vi "Register.vi"(4 "line limit":i32, 6 "log limit":i32, 8 "error in (no error)":errorcluster, 9 "auto-scroll":bool, 10 "ctl ref":refnum<vi>, 11 "handler name":string) -> (0 "error out":errorcluster)   [LabVIEW 2018, in "GLog.lvlib" / "UI Updater.lvlib"]
uses:
  UI Updater.lvlib
  UI Updater.vi
  UI Updater Global.vi
panel:
  # "Connector Pane"
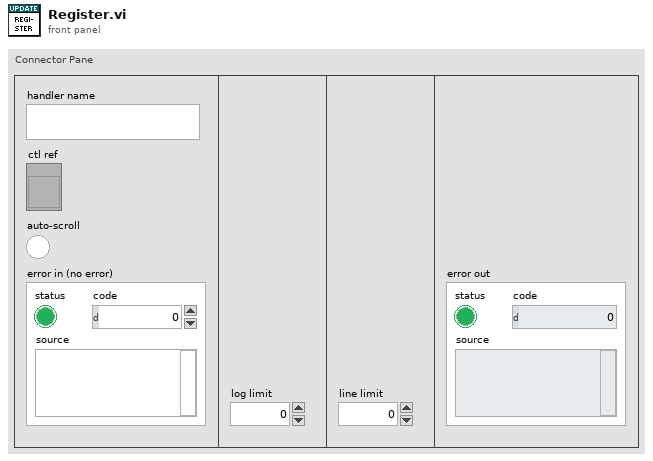
[diagram p1: front panel]
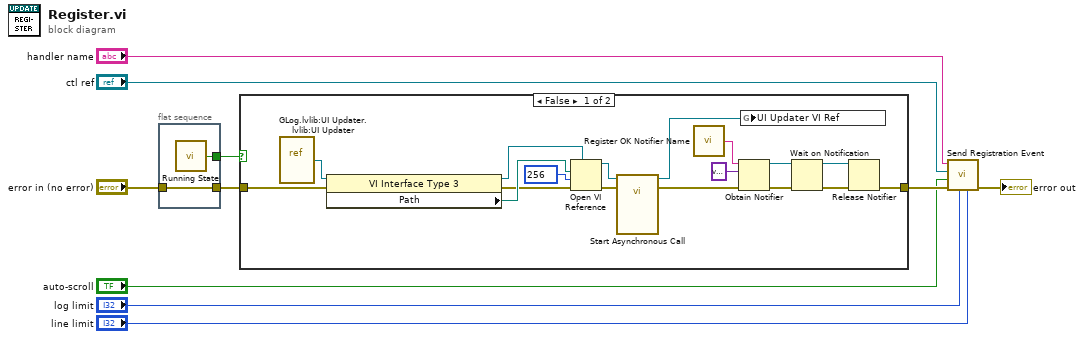
[diagram p0: block diagram]
diagram:
  n1 = flat-sequence {
    tunnel: [w12] -> w10
    tunnel: [w11] -> w2
    tunnel: "error in (no error)" -> [w11]
    frame #0 {
      n2 = call "Running State.vi"() -> ("Running?"=w12:bool)  [unwired: 1 in]
    }
  }
  n3 = case shown="False" w10 {
    tunnel: [w15 w30] -> w9
    tunnel: w2 -> [w22 w30]
    frame False {
      n4 = vi-ref "GLog.lvlib:UI Updater.lvlib:UI Updater.vi"() -> (w27:refnum<vi>)
      n5 = property class="VI Interface Type 3"(reference=w27, error in=w22) -> (reference out=w26:refnum<vi>, error out=w23:errorcluster, "Path"=w28:path)
      n6 = Open VI Reference(type specifier VI Refnum (for type only)=w26, vi path=w28, options=256, error in (no error)=w23) -> (vi reference=w29:refnum<vi>, error out=w24:errorcluster)  [unwired: 2 in]
      n7 = call-by-ref "Start Asynchronous Call"(reference=w29, error in=w24) -> (reference out=w13:refnum<vi>, error out=w19:errorcluster)  [unwired: 12 in]
      n8 = call "Register OK Notifier Name.vi"() -> ("register ok notifier"=w21:string)  [unwired: 1 in]
      n9 = Obtain Notifier(name (unnamed)=w21, notification data type=variant, error in (no error)=w19) -> (notifier out=w17:refnum<notifier>, error out=w18:errorcluster)  [unwired: 1 in, 1 out]
      n10 = global write "UI Updater Global.vi" "UI Updater VI Ref"(w13) -> ()
      n11 = Wait on Notification(notifier=w17, error in (no error)=w18) -> (notifier out=w14:refnum<notifier>, error out=w16:errorcluster)  [unwired: 2 in, 2 out]
      n12 = Release Notifier(notifier=w14, error in (no error)=w16) -> (error out=w15:errorcluster)  [unwired: 1 in, 2 out]
    }
    frame True {
    }
  }
  n13 = call "Send Registration Event.vi"("line limit"="line limit", "log limit"="log limit", "error in (no error)"=w9, "auto-scroll"="auto-scroll", "ctl ref"="ctl ref", "handler name"="handler name") -> ("error out"=→"error out":errorcluster)  [unwired: 5 in]
